vi "Assign Pixel to Wing Sector (FPGA).vi"(4 "End of Data?":bool, 6 "Valid Data?":bool, 7 "Pixel Intensity In":u8, 8 "Right Wing?":bool, 9 "Sector Parameters":T1, 10 "Pixel Y":u16, 11 "Pixel X":u16) -> (1 "Pixel Intensity Out":u8, 2 "sector #":u8, 3 "output valid":bool)   [LabVIEW 2013]
uses:
  Sector Parameter Cluster.ctl
  <vilib>/rvi/FXPMathLib/FxpRectToPolar/XNode/nifxpmath_RectToPolar.xnode
  <vilib>/rvi/FXPMathLib/FxpSub/XNode/nifxpmath_Sub.xnode
  <vilib>/rvi/FXPMathLib/sim/FxpSim.dll
  <vilib>/rvi/FXPMathLib/FxpAdd/XNode/nifxpmath_Add.xnode
  <vilib>/rvi/FXPMathLib/FxpDiv/XNode/nifxpmath_Div.xnode
  <vilib>/rvi/FXPMathLib/FxpRectToPolar/simVIs/DllFxpRectToPolarTemp_sub.vi
  <vilib>/rvi/FXPMathLib/FxpRectToPolar/subVIs/nifxpmath_RectToPolar_SimConfig.ctl
  <vilib>/ptbypt/NI_PtbyPt.lvlib
  <vilib>/rvi/FXPMathLib/FxpDiv/simVIs/DllFxpDivTemp_sub.vi
  <vilib>/rvi/FXPMathLib/FxpDiv/subVIs/nifxpmath_Div_SimConfig.ctl
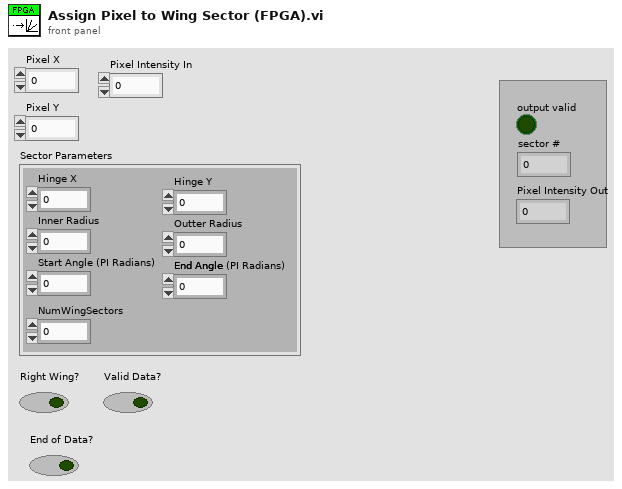
[diagram p1: front panel]
types:
  T1 = typedef "Sector Parameter Cluster.ctl" = cluster{"Start Angle":fxp<+/-,17,2>, "End Angle":fxp<+/-,17,2>, "Inner Radius":u16, "Outter Radius":u16, "Hinge X":u16, "Hinge Y":u16, "NumWingSectors":u8}
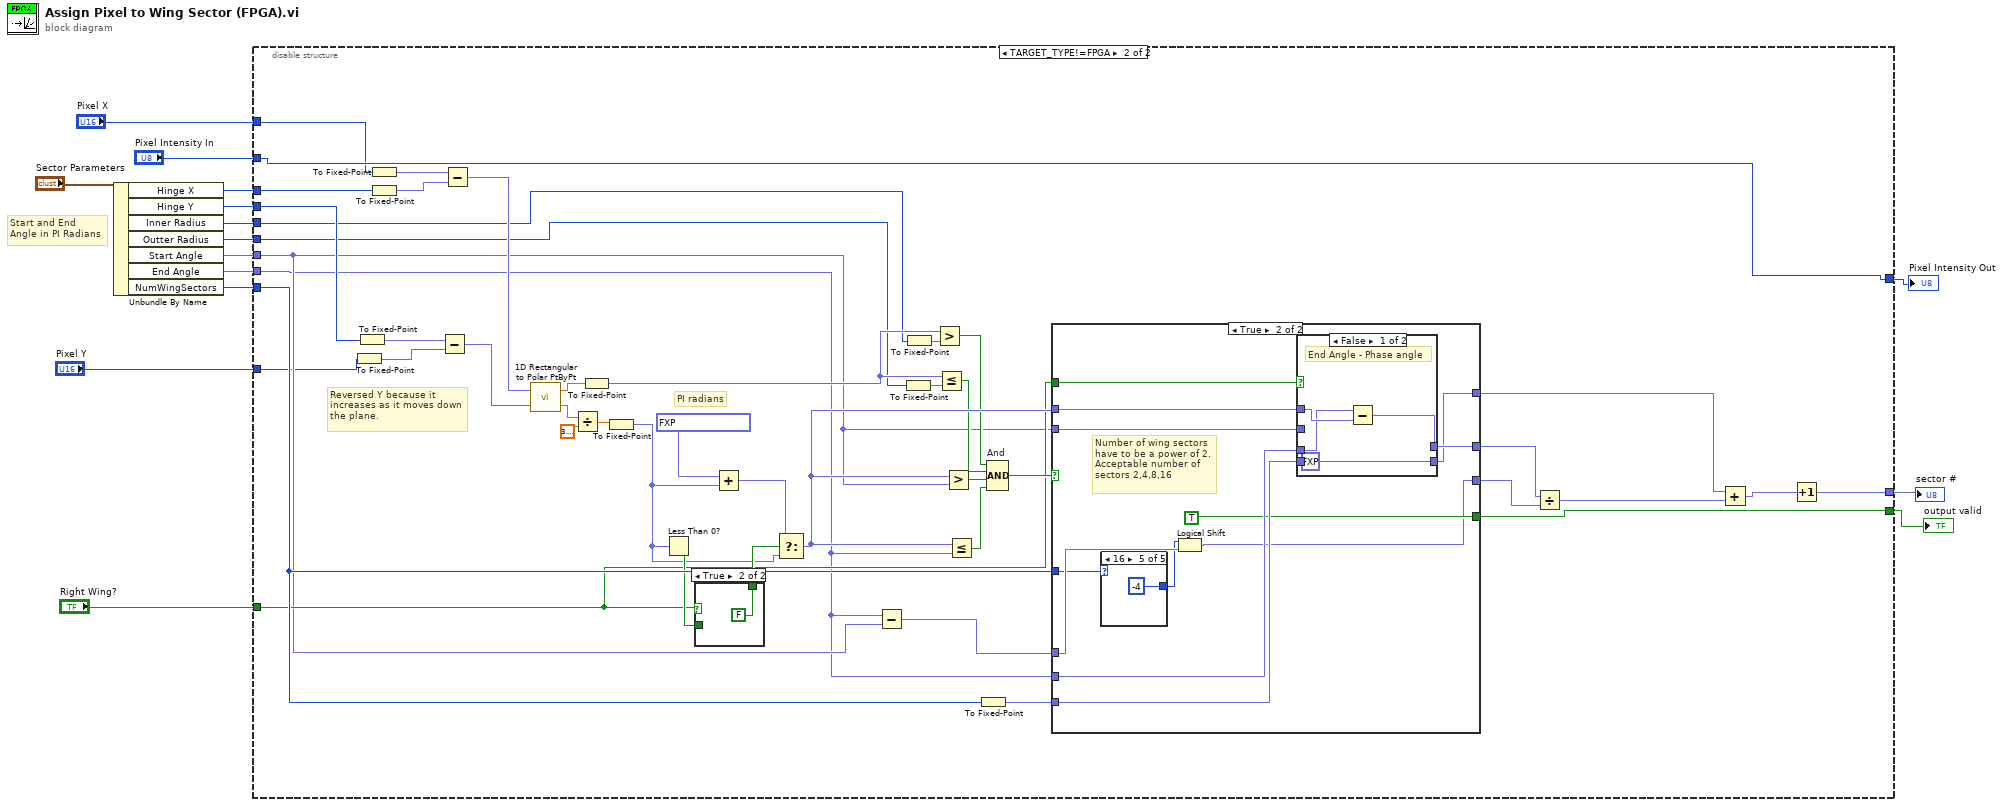
[diagram p0: block diagram]
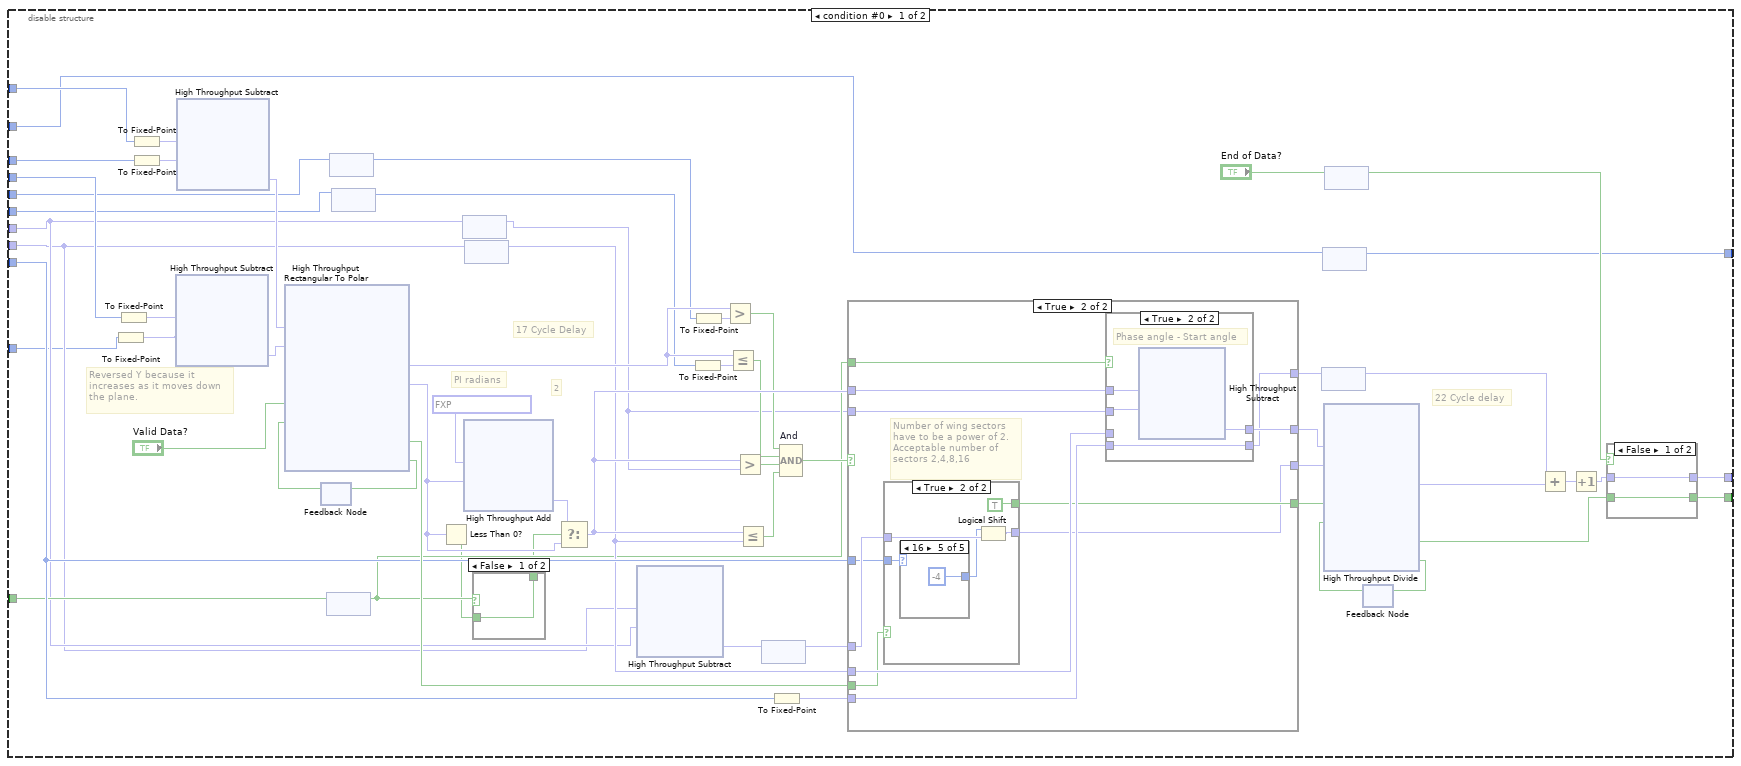
[diagram p2: hidden frame]
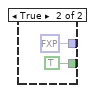
[diagram p3: hidden frame]
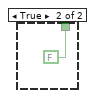
[diagram p4: hidden frame]
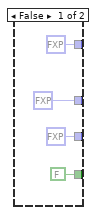
[diagram p5: hidden frame]
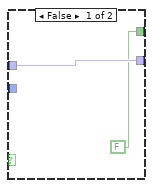
[diagram p6: hidden frame]
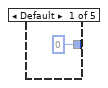
[diagram p7: hidden frame]
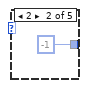
[diagram p8: hidden frame]
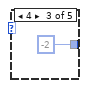
[diagram p9: hidden frame]
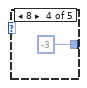
[diagram p10: hidden frame]
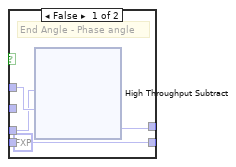
[diagram p11: hidden frame]
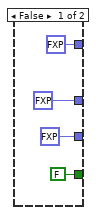
[diagram p13: hidden frame]
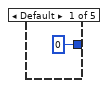
[diagram p14: hidden frame]
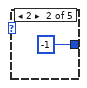
[diagram p15: hidden frame]
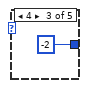
[diagram p16: hidden frame]
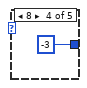
[diagram p17: hidden frame]
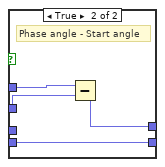
[diagram p18: hidden frame]
diagram:
  # "Start and End\nAngle in PI Radians"
  n1 = Unbundle By Name("Sector Parameters") -> ("Hinge X"=w13:u16, "Hinge Y"=w15:u16, "Inner Radius"=w11:u16, "Outter Radius"=w10:u16, "Start Angle"=w8:fxp<+/-,17,2>, "End Angle"=w7:fxp<+/-,17,2>, "NumWingSectors"=w14:u8)
  n2 = disable-structure shown="TARGET_TYPE!=FPGA" {
    disable-tunnel: w15 -> [w60 w218]
    disable-tunnel: w14 -> [w46 w210]
    disable-tunnel: w13 -> [w45 w209]
    disable-tunnel: w11 -> [w44 w198]
    disable-tunnel: w10 -> [w42 w197]
    disable-tunnel: "Right Wing?" -> [w36 w199]
    disable-tunnel: w8 -> [w33 w196]
    disable-tunnel: w7 -> [w31 w195]
    disable-tunnel: [w25 w186] -> w6
    disable-tunnel: [w23 w190] -> w5
    disable-tunnel: "Pixel X" -> [w21 w192]
    disable-tunnel: "Pixel Y" -> [w20 w191]
    disable-tunnel: [w19 w193] -> w2
    disable-tunnel: "Pixel Intensity In" -> [w18 w193]
    frame condition #0 {
      # "17 Cycle Delay"
      # "Reversed Y because it\nincreases as it moves down\nthe plane."
      # "PI radians"
      # "22 Cycle delay"
      # "2"
      n3 = To Fixed-Point(number=w20) -> (fixed-point=w50:fxp<+,11,11>)  [unwired: 1 in]
      n4 = To Fixed-Point(number=w60) -> (fixed-point=w51:fxp<+,11,11>)  [unwired: 1 in]
      n5 = To Fixed-Point(number=w21) -> (fixed-point=w49:fxp<+,11,11>)  [unwired: 1 in]
      n6 = To Fixed-Point(number=w45) -> (fixed-point=w48:fxp<+,11,11>)  [unwired: 1 in]
      n7 = xnode "High Throughput Subtract"("x"=w51, "y"=w50) -> ("x-y"=w59:fxp<+/-,12,12>)
      n8 = xnode "High Throughput Subtract"("x"=w49, "y"=w48) -> ("x-y"=w58:fxp<+/-,12,12>)
      n9 = feedback #1() -> (w65:bool)  [unwired: 1 in]
      n10 = xnode "High Throughput Rectangular To Polar"("x"=w58, "y"=w59, "input valid"="Valid Data?", "ready for output (T)"=w65) -> ("magnitude"=w73:fxp<+,12,12>, "phase (pi)"=w70:fxp<+/-,16,2>, "output valid"=w47:bool, "ready for input"=w66:bool)
      n11 = feedback-in #1(w66) -> ()
      n12 = feedback #2() -> (w39:bool)  [unwired: 1 in]
      n13 = feedback-in #2(w36) -> ()
      n14 = feedback #3() -> (w43:u16)  [unwired: 1 in]
      n15 = feedback-in #3(w44) -> ()
      n16 = feedback #4() -> (w41:u16)  [unwired: 1 in]
      n17 = feedback-in #4(w42) -> ()
      n18 = Less Than 0?(x=w70) -> (x < 0?=w37:bool)
      n19 = feedback #5() -> (w32:fxp<+/-,17,2>)  [unwired: 1 in]
      n20 = feedback-in #5(w33) -> ()
      n21 = xnode ("High Throughput Add")("x"=fxp<+/-,16,2> 1.99993896484375 ("y"), "y"=w70) -> ("x+y"=w69:fxp<+/-,17,3>)
      n22 = feedback #6() -> (w40:fxp<+/-,17,2>)  [unwired: 1 in]
      n23 = feedback-in #6(w31) -> ()
      n24 = case shown="False" w39 {
        tunnel: [w79 FALSE ("s")] -> w38
        tunnel: w37 -> [w79 _]
        frame False {
        }
        frame True {
        }
      }
      n25 = Select(t=w69, s=w38, f=w70) -> (s? t:f=w67:fxp<+/-,17,3>)
      n26 = xnode ("High Throughput Subtract")("x"=w31, "y"=w33) -> ("x-y"=w30:fxp<+/-,18,3>)
      n27 = To Fixed-Point(number=w41) -> (fixed-point=w72:fxp<+,16,16>)  [unwired: 1 in]
      n28 = To Fixed-Point(number=w43) -> (fixed-point=w74:fxp<+,16,16>)  [unwired: 1 in]
      n29 = Greater?(x=w73, y=w74) -> (0:w64:bool)
      n30 = Less Or Equal?(x=w73, y=w72) -> (x <= y?=w63:bool)
      n31 = Greater?(x=w67, y=w32) -> (0:w62:bool)
      n32 = Less Or Equal?(x=w67, y=w40) -> (x <= y?=w61:bool)
      n33 = feedback #7() -> (w29:fxp<+/-,18,3>)  [unwired: 1 in]
      n34 = feedback-in #7(w30) -> ()
      n35 = To Fixed-Point(number=w46) -> (fixed-point=w35:fxp<+,8,8>)  [unwired: 1 in]
      n36 = Compound Arithmetic op=AND "And"(w64, w63, w62, w61) -> (w71:bool)
      n37 = case shown="True" w71 {
        tunnel: w67 -> [_ w125]
        tunnel: w32 -> [_ w124]
        tunnel: [fxp<+/-,18,3> 0.0 ("x-y") w115] -> w55
        tunnel: w40 -> [_ w122]
        tunnel: w35 -> [_ w123]
        tunnel: [fxp<+/-,20,5> 0.0 ("x-y") w121] -> w56
        tunnel: [FALSE ("output valid") w116] -> w54
        tunnel: [fxp<+,8,8> 0.0 w120] -> w52
        tunnel: w29 -> [_ w119]
        tunnel: w47 -> [_ w118]
        tunnel: w46 -> [_ w117]
        tunnel: w39 -> [_ w114]
        frame False {
        }
        frame True {
          # "Number of wing sectors\nhave to be a power of 2.\nAcceptable number of\nsectors 2,4,8,16"
          n38 = case shown="True" w118 {
            tunnel: w117 -> [_ w132]
            tunnel: w119 -> [w127 w131]
            tunnel: [w127 w129] -> w115
            tunnel: [FALSE ("output valid") TRUE ("output valid")] -> w116
            frame False {
            }
            frame True {
              n39 = case shown="16" w132 {
                tunnel: [i16 0 ("y") i16 -1 ("y") i16 -2 ("y") i16 -3 ("y") i16 -4 ("y")] -> w130
                frame Default {
                }
                frame 2 {
                }
                frame 4 {
                }
                frame 8 {
                }
                frame 16 {
                }
              }
              n40 = Logical Shift(y=w130, x=w131) -> (x << y=w129:fxp<+/-,18,3>)
            }
          }
          n41 = case shown="True" w114 {
            tunnel: w125 -> [w140 w145]
            tunnel: w124 -> [_ w144]
            tunnel: [w141 w143] -> w121
            tunnel: w123 -> [_ w142]
            tunnel: [fxp<+,8,8> 0.0 w142] -> w120
            tunnel: w122 -> [w139 _]
            frame False {
              # "End Angle - Phase angle"
              n42 = xnode "High Throughput Subtract"("x"=w139, "y"=w140) -> ("x-y"=w141:fxp<+/-,19,4>)
            }
            frame True {
              # "Phase angle - Start angle"
              n43 = xnode ("High Throughput Subtract")("x"=w145, "y"=w144) -> ("x-y"=w143:fxp<+/-,19,4>)
            }
          }
        }
      }
      n44 = feedback #8() -> (w34:fxp<+,8,8>)  [unwired: 1 in]
      n45 = feedback-in #8(w52) -> ()
      n46 = feedback #9() -> (w19:u8)  [unwired: 1 in]
      n47 = feedback-in #9(w18) -> ()
      n48 = feedback #10() -> (w26:bool)  [unwired: 1 in]
      n49 = feedback-in #10("End of Data?") -> ()
      n50 = feedback #11() -> (w53:bool)  [unwired: 1 in]
      n51 = xnode "High Throughput Divide"("x"=w56, "y"=w55, "input valid"=w54, "ready for output (T)"=w53) -> ("x/y"=w17:fxp<+/-,20,20>, "output valid"=w22:bool, "ready for input"=w57:bool)
      n52 = feedback-in #11(w57) -> ()
      n53 = Add(x=w34, y=w17) -> (x+y=w24:fxp<+/-,21,21>)
      n54 = Increment(x=w24) -> (x+1=w16:fxp<+/-,21,21>)
      n55 = case shown="False" w26 {
        tunnel: [w76 fxp<+/-,17,17> 0.0] -> w25
        tunnel: w16 -> [w76 _]
        tunnel: [w75 TRUE ("output valid")] -> w23
        tunnel: w22 -> [w75 _]
        frame False {
        }
        frame True {
        }
      }
    }
    frame condition #1 (active) {
      # "Reversed Y because it\nincreases as it moves down\nthe plane."
      # "PI radians"
      n56 = To Fixed-Point(number=w191) -> (fixed-point=w213:fxp<+,11,11>)  [unwired: 1 in]
      n57 = To Fixed-Point(number=w218) -> (fixed-point=w214:fxp<+,11,11>)  [unwired: 1 in]
      n58 = To Fixed-Point(number=w192) -> (fixed-point=w212:fxp<+,11,11>)  [unwired: 1 in]
      n59 = To Fixed-Point(number=w209) -> (fixed-point=w211:fxp<+,11,11>)  [unwired: 1 in]
      n60 = Subtract(x=w214, y=w213) -> (x-y=w217:fxp<+/-,12,12>)
      n61 = Subtract(x=w212, y=w211) -> (x-y=w216:fxp<+/-,12,12>)
      n62 = call <vilib>:"1D Rectangular to Polar PtByPt.vi"("y"=w217, "x"=w216) -> ("phase"=w203:dbl, "magnitude"=w205:dbl)
      n63 = Divide(x=w203, y=3.141592653589793) -> (x/y=w201:dbl)
      n64 = To Fixed-Point(number=w205) -> (fixed-point=w204:fxp<+,12,12>)  [unwired: 1 in]
      n65 = To Fixed-Point(number=w201) -> (fixed-point=w200:fxp<+/-,16,2>)  [unwired: 1 in]
      n66 = Less Than 0?(x=w200) -> (x < 0?=w207:bool)
      n67 = case shown="True" w199 {
        tunnel: [w229 FALSE ("s")] -> w208
        tunnel: w207 -> [w229 _]
        frame False {
        }
        frame True {
        }
      }
      n68 = Add(x=fxp<+/-,16,2> 1.99993896484375 ("y"), y=w200) -> (x+y=w225:fxp<+/-,17,3>)
      n69 = Select(t=w225, s=w208, f=w200) -> (s? t:f=w223:fxp<+/-,17,3>)
      n70 = Subtract(x=w195, y=w196) -> (x-y=w194:fxp<+/-,18,3>)
      n71 = To Fixed-Point(number=w197) -> (fixed-point=w227:fxp<+,16,16>)  [unwired: 1 in]
      n72 = To Fixed-Point(number=w198) -> (fixed-point=w228:fxp<+,16,16>)  [unwired: 1 in]
      n73 = Greater?(x=w204, y=w228) -> (0:w222:bool)
      n74 = Less Or Equal?(x=w204, y=w227) -> (x <= y?=w221:bool)
      n75 = Greater?(x=w223, y=w196) -> (0:w220:bool)
      n76 = Less Or Equal?(x=w223, y=w195) -> (x <= y?=w219:bool)
      n77 = To Fixed-Point(number=w210) -> (fixed-point=w206:fxp<+,8,8>)  [unwired: 1 in]
      n78 = Compound Arithmetic op=AND "And"(w222, w221, w220, w219) -> (w226:bool)
      n79 = case shown="True" w226 {
        tunnel: w223 -> [_ w246]
        tunnel: w196 -> [_ w245]
        tunnel: [fxp<+/-,18,3> 0.0 ("x-y") w237] -> w188
        tunnel: w195 -> [_ w243]
        tunnel: w206 -> [_ w244]
        tunnel: [fxp<+/-,20,5> 0.0 ("x-y") w242] -> w215
        tunnel: [FALSE ("output valid") TRUE ("output valid")] -> w190
        tunnel: [fxp<+,8,8> 0.0 w241] -> w189
        tunnel: w194 -> [_ w240]
        tunnel: w210 -> [_ w239]
        tunnel: w199 -> [_ w236]
        frame False {
        }
        frame True {
          # "Number of wing sectors\nhave to be a power of 2.\nAcceptable number of\nsectors 2,4,8,16"
          n80 = case shown="16" w239 {
            tunnel: [i16 0 ("y") i16 -1 ("y") i16 -2 ("y") i16 -3 ("y") i16 -4 ("y")] -> w235
            frame Default {
            }
            frame 2 {
            }
            frame 4 {
            }
            frame 8 {
            }
            frame 16 {
            }
          }
          n81 = Logical Shift(y=w235, x=w240) -> (x << y=w237:fxp<+/-,18,3>)
          n82 = case shown="False" w236 {
            tunnel: w246 -> [w254 w259]
            tunnel: w245 -> [_ w258]
            tunnel: [w255 w257] -> w242
            tunnel: w244 -> [_ w256]
            tunnel: [fxp<+,8,8> 0.0 w256] -> w241
            tunnel: w243 -> [w253 _]
            frame False {
              # "End Angle - Phase angle"
              n83 = Subtract(x=w253, y=w254) -> (x-y=w255:fxp<+/-,19,4>)
            }
            frame True {
              # "Phase angle - Start angle"
              n84 = Subtract(x=w259, y=w258) -> (x-y=w257:fxp<+/-,19,4>)
            }
          }
        }
      }
      n85 = Divide(x=w215, y=w188) -> (x/y=w185:fxp<+/-,20,20>)
      n86 = Add(x=w189, y=w185) -> (x+y=w187:fxp<+/-,21,21>)
      n87 = Increment(x=w187) -> (x+1=w186:fxp<+/-,21,21>)
    }
  }
  "output valid" <- w5
  "sector #" <- w6
  "Pixel Intensity Out" <- w2
